vi "VIH Project Tree - Find File in Project Tree.vi"(6 "Ena <Invalid> (F)":bool, 8 "error in":errorcluster, 10 "File Path":path, 11 "Project Tree":T1) -> (0 "error out":errorcluster, 1 "Tree Item Tags (Dynamic)":string[](array[string]), 2 "Tree Item Tag (Static)":string, 3 "dup Project Tree":T1)   [LabVIEW 2014]
doc: "::: VI Helpeks :::\nCopyright (c) 2000-2026 Konstantin Shifershteyn. All rights reserved."
uses:
  VIH Project Tree Typedef - Tree Refnum.ctl
  VIH Project Tree Typedef - Tree Item Type.ctl
panel:
  # "VI Helpeks\nCopyright (c) 2012-2026 Konstantin Shifershteyn"
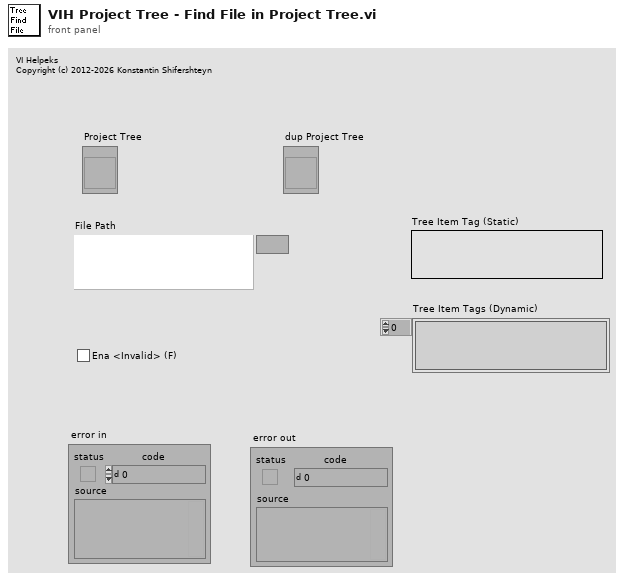
[diagram p1: front panel]
types:
  T1 = typedef "VIH Project Tree Typedef - Tree Refnum.ctl" = refnum<vi>
  T2 = typedef "VIH Project Tree Typedef - Tree Item Type.ctl" = enum32{"<Invalid>", "Project", "Proj Files", "Proj Rules", "File Group", "Rule Group", "Any File", "LV Func", ".mnu", ".mnu (dyn)", ".vi", ".vi (dyn)", ".vit", ".vit (dyn)", ".ctl", ".ctl (dyn)", ".ctt", ".ctt (dyn)", "polyVI", "polyVI (dyn)", "expVI", "expVI (dyn)", "HTML", "PolyVI Inst"}
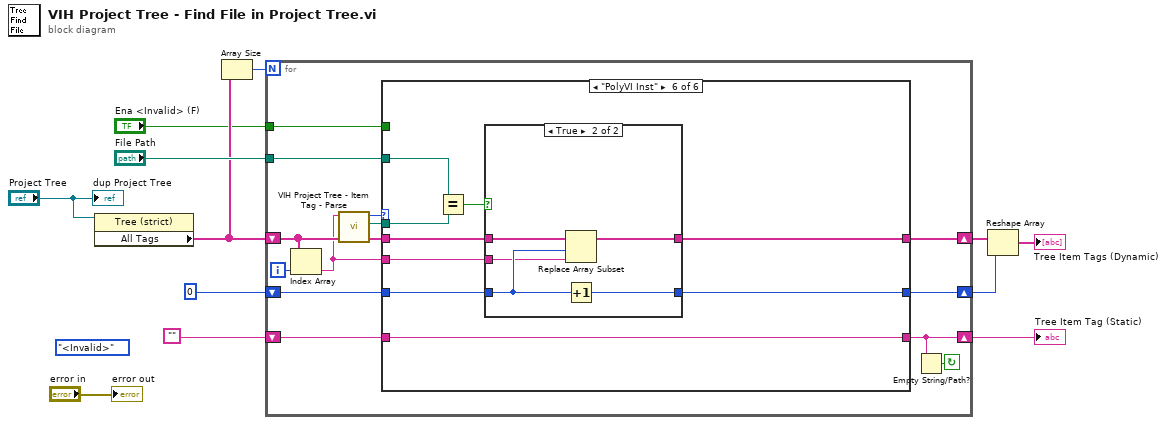
[diagram p0: block diagram]
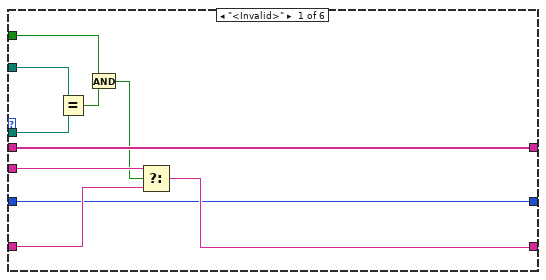
[diagram p2: hidden frame]
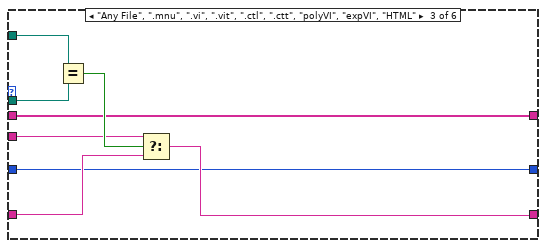
[diagram p4: hidden frame]
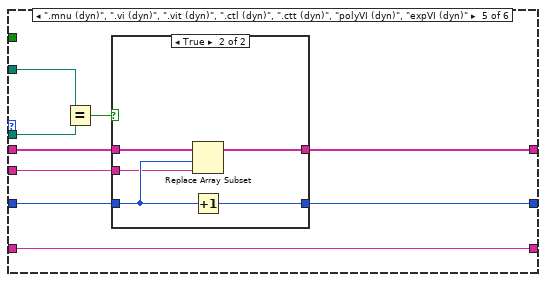
[diagram p6: hidden frame]
diagram:
  (unwired) VIH_Project_Tree_Typedef_-_Tree_Item_Type."<Invalid>" ("Item Type")
  n1 = property class="Tree (strict)"(reference="Project Tree") -> ("All Tags"=w2:string[])  [unwired: 1 in, 2 out]
  n2 = Array Size(array=w2) -> (size(s)=w3:i32)
  n3 = for {
    N: w3 -> [_]
    shift-right: [w21] -> w9
    shift-left: "" -> [w24]
    shift-right: [w20] -> w6
    shift-left: w2 -> [w15]
    tunnel: "File Path" -> [w22]
    shift-right: [w18] -> w5
    shift-left: 0 -> [w17]
    tunnel: "Ena <Invalid> (F)" -> [w13]
    i -> [w16]
    stop <- w19 continue-if-true
    n4 = Index Array(array=w15, index=w16) -> (element=w14:string)
    n5 = call "VIH Project Tree - Item Tag - Parse.vi"("Tree Item Tag"=w14) -> ("Item File Path"=w23:path, "Item Type"=w25:T2)  [unwired: 8 in, 1 out]
    n6 = case shown="\"PolyVI Inst\"" w25 {
      tunnel: [w33 w38 w43 w49 w58 w74] -> w21
      tunnel: w24 -> [w34 w38 w44 w49 w58 w74]
      tunnel: [w32 w37 w42 w48 w53 w69] -> w20
      tunnel: w15 -> [w32 w37 w42 w48 w56 w72]
      tunnel: w23 -> [w29 _ w39 _ w50 w66]
      tunnel: w22 -> [w30 _ w40 _ w51 w67]
      tunnel: w14 -> [w35 _ w45 _ w52 w68]
      tunnel: [w31 w36 w41 w47 w55 w71] -> w18
      tunnel: w17 -> [w31 w36 w41 w47 w54 w70]
      tunnel: w13 -> [w28 _ _ _ _ _]
      frame "<Invalid>" {
        n7 = Equal?(x=w30, y=w29) -> (x = y?=w27:bool)
        n8 = And(x=w28, y=w27) -> (x .and. y?=w26:bool)
        n9 = Select(t=w35, s=w26, f=w34) -> (s? t:f=w33:string)
      }
      frame "Project".."Rule Group" {
      }
      frame "Any File", ".mnu", ".vi", ".vit", ".ctl", ".ctt", "polyVI", "expVI", "HTML" {
        n10 = Equal?(x=w40, y=w39) -> (x = y?=w46:bool)
        n11 = Select(t=w45, s=w46, f=w44) -> (s? t:f=w43:string)
      }
      frame "LV Func" {
      }
      frame ".mnu (dyn)", ".vi (dyn)", ".vit (dyn)", ".ctl (dyn)", ".ctt (dyn)", "polyVI (dyn)", "expVI (dyn)" {
        n12 = Equal?(x=w51, y=w50) -> (x = y?=w57:bool)
        n13 = case shown="True" w57 {
          tunnel: w56 -> [w60 w64]
          tunnel: [w59 w65] -> w55
          tunnel: w54 -> [w59 w63]
          tunnel: [w60 w62] -> w53
          tunnel: w52 -> [_ w61]
          frame False {
          }
          frame True {
            n14 = Replace Array Subset(array=w64, new element=w61, index=w63) -> (w62:string[])
            n15 = Increment(x=w63) -> (x+1=w65:i32)
          }
        }
      }
      frame "PolyVI Inst" {
        n16 = Equal?(x=w67, y=w66) -> (x = y?=w73:bool)
        n17 = case shown="True" w73 {
          tunnel: w72 -> [w76 w80]
          tunnel: [w75 w81] -> w71
          tunnel: w70 -> [w75 w79]
          tunnel: [w76 w78] -> w69
          tunnel: w68 -> [_ w77]
          frame False {
          }
          frame True {
            n18 = Replace Array Subset(array=w80, new element=w77, index=w79) -> (w78:string[])
            n19 = Increment(x=w79) -> (x+1=w81:i32)
          }
        }
      }
    }
    n20 = Empty String/Path?(string/path=w21) -> (empty?=w19:bool)
  }
  "Tree Item Tag (Static)" <- w9
  n21 = Reshape Array(w6, w5) -> (→"Tree Item Tags (Dynamic)":string[])
  "dup Project Tree" <- "Project Tree"
  "error out" <- "error in"
